vi "Update Value.vi"(6 "Time":dbl, 8 "error in (no error)":errorcluster, 11 "ImageButtonControl in":refnum<class "ImageButtonControl.lvclass">) -> (0 "error out":errorcluster, 1 "Update":bool, 2 "Value":variant, 3 "ImageButtonControl out":refnum<class "ImageButtonControl.lvclass">)   [LabVIEW 2020, in "VolatusGUIElements.lvlib" / "ImageButtonControl.lvclass"]
uses:
  ImageButtonControl.lvclass
  ImageButtonControl.lvclass/ImageButtonControl.ctl
  lv-vecto/Vecto/Channel DBL/Channel DBL.lvclass/Channel DBL.ctl
  lv-vecto/Vecto/Group DBL/Value by Index.vi
  lv-vecto/Vecto/Channel DBL/Channel DBL.lvclass
  lv-vecto/Vecto/Vecto.lvlib
  VolatusGUI/Element Inhibit/Element Inhibit.lvclass
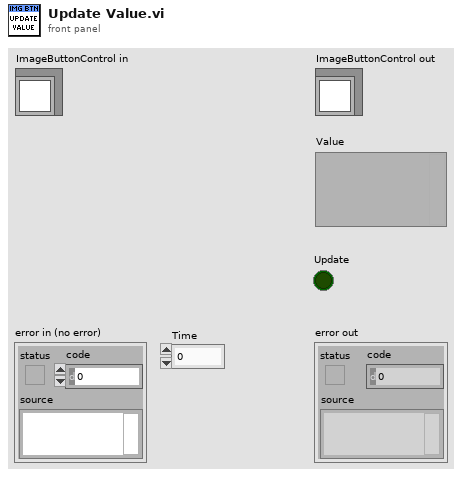
[diagram p1: front panel]
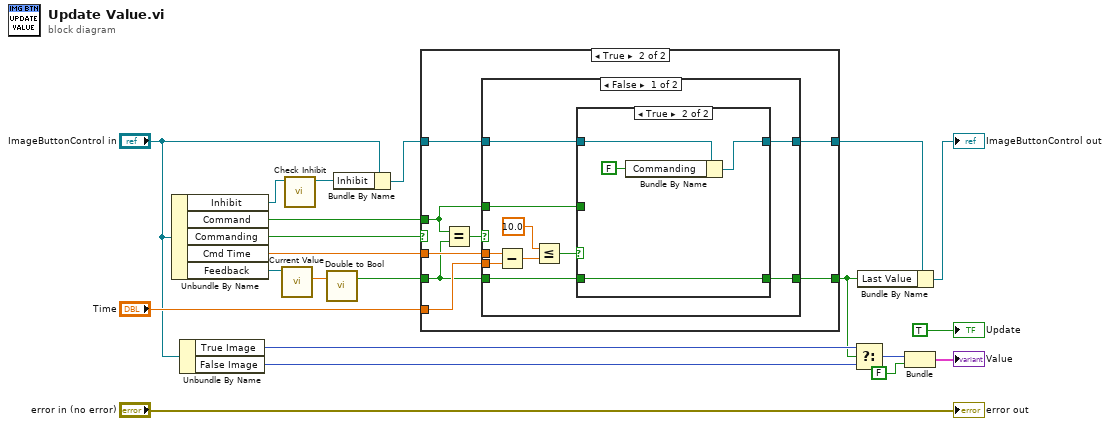
[diagram p0: block diagram]
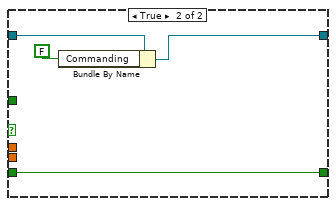
[diagram p4: hidden frame]
diagram:
  n1 = Unbundle By Name("ImageButtonControl in") -> ("Inhibit"=w3:refnum<class "Element Inhibit.lvclass">, "Command"=w16:bool, "Commanding"=w20:bool, "Cmd Time"=w18:dbl, "Feedback"=w21:refnum<class "Channel DBL.lvclass">)
  n2 = Unbundle By Name("ImageButtonControl in") -> ("True Image"=w9:picture, "False Image"=w8:picture)
  n3 = call "Current Value.vi"("Channel in"=w21) -> ("Scaled"=w19:dbl)  [unwired: 6 in, 4 out]
  n4 = call "Check Inhibit.vi"("Element Inhibit in"=w3) -> ("Element Inhibit out"=w1:refnum<class "Element Inhibit.lvclass">)  [unwired: 9 in, 1 out]
  n5 = call "Double to Bool.vi"("Double"=w19) -> ("Bool"=w17:bool)  [unwired: 2 in]
  n6 = Bundle By Name(cluster="ImageButtonControl in", "Inhibit"=w1) -> (w2:refnum<class "ImageButtonControl.lvclass">)
  n7 = case shown="True" w20 {
    tunnel: w17 -> [w23 w28]
    tunnel: w18 -> [_ w31]
    tunnel: "Time" -> [_ w30]
    tunnel: w16 -> [_ w24]
    tunnel: w2 -> [w22 w27]
    tunnel: [w22 w26] -> w15
    tunnel: [w23 w25] -> w4
    frame False {
    }
    frame True {
      n8 = Equal?(x=w24, y=w28) -> (x = y?=w29:bool)
      n9 = case shown="False" w29 {
        tunnel: w31 -> [w41 _]
        tunnel: w30 -> [w40 _]
        tunnel: w28 -> [w34 w48]
        tunnel: w27 -> [w36 w51]
        tunnel: [w35 w49] -> w26
        tunnel: [w32 w48] -> w25
        tunnel: w24 -> [w33 _]
        frame False {
          n10 = Subtract(x=w41, y=w40) -> (x-y=w39:dbl)
          n11 = Less Or Equal?(x=10.0, y=w39) -> (x <= y?=w37:bool)
          n12 = case shown="True" w37 {
            tunnel: w36 -> [w42 w47]
            tunnel: [w42 w45] -> w35
            tunnel: w34 -> [_ w44]
            tunnel: w33 -> [w43 _]
            tunnel: [w43 w44] -> w32
            frame False {
            }
            frame True {
              n13 = Bundle By Name(cluster=w47, "Commanding"=FALSE) -> (w45:refnum<class "ImageButtonControl.lvclass">)
            }
          }
        }
        frame True {
          n14 = Bundle By Name(cluster=w51, "Commanding"=FALSE) -> (w49:refnum<class "ImageButtonControl.lvclass">)
        }
      }
    }
  }
  n15 = Select(t=w9, s=w4, f=w8) -> (s? t:f=w7:picture)
  n16 = Bundle By Name(cluster=w15, "Last Value"=w4) -> (→"ImageButtonControl out":refnum<class "ImageButtonControl.lvclass">)
  n17 = Bundle("False Image"=w7, FALSE) -> (→"Value":cluster{"False Image":picture, bool})  [unwired: 1 in]
  "error out" <- "error in (no error)"
  "Update" <- TRUE ("Update")
